vi "measure BT Min Freq.vi"(8 "error in (no error)":errorcluster, 10 "Threshold Level":dbl, 11 "SA Measurement in":refnum<class "SA Measurement.lvclass">) -> (0 "error out":errorcluster, 3 "SA Measurement out":refnum<class "SA Measurement.lvclass">)   [LabVIEW 2023, in "Spectrum Analyzer.lvlib" / "SA Measurement.lvclass"]
uses:
  SA Measurement.lvclass
  SA Measurement.lvclass/SA Measurement.ctl
  TYPE DEFINITION/Keysight 9020A/TYPE Measurement Preset.ctl
  Spectrum Analyzer.lvlib
  TYPE DEFINITION/TYPE RBW and VBW Select.ctl
  Interface_Spectrum/Interface_Spectrum.lvclass
  <vilib>/Utility/file.llb/Read Delimited Spreadsheet (string).vi
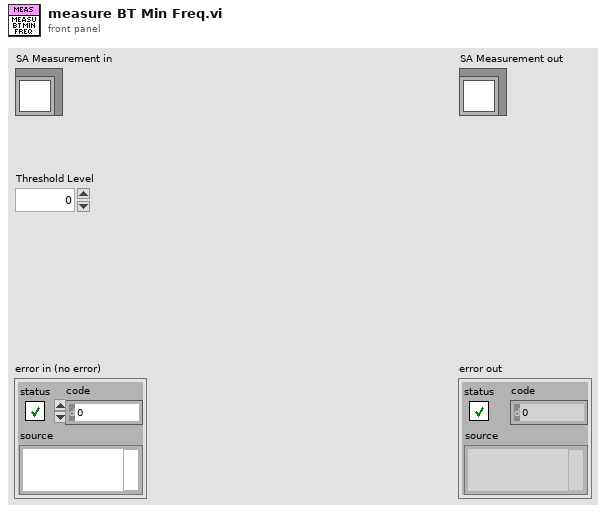
[diagram p1: front panel]
types:
  T1 = typedef "Spectrum Analyzer.lvlib/TYPE RBW and VBW Select.ctl" = enum16{"Res BW", "Video BW"}
  T2 = typedef "Spectrum Analyzer.lvlib/TYPE Measurement Preset.ctl" = enum16{"Sweep SA Mode", "Channel Power", "Occupied BW", "ACP", "Spurious Emission", "Spurious Emission Mask", "Burst Power (Transmit Power)"}
  T3 = typedef "Spectrum Analyzer.lvlib/TYPE Reference Level and Atten Param.ctl" = cluster{"Reference Level":dbl, "Atten":i32, "Atten Auto?":bool, "Reference Level Offset":dbl}
  T4 = typedef "Spectrum Analyzer.lvlib/TYPE Display Trace Mode Select.ctl" = enum16{"Clear Write", "Max Hold", "Min Hold", "Average", "View"}
  T5 = typedef "Spectrum Analyzer.lvlib/TYPE Detect Mode Select.ctl" = enum16{"Det Auto (Normal)", "Auto Peak", "Positive Peak", "Negative Peak", "Sample", "RMS", "Average", "Quasipeak", "CISPR Average", "RMS Average"}
  T6 = cluster{"Trace Mode":T4, "Detector Type":T5, "Detect Auto?":bool}[]
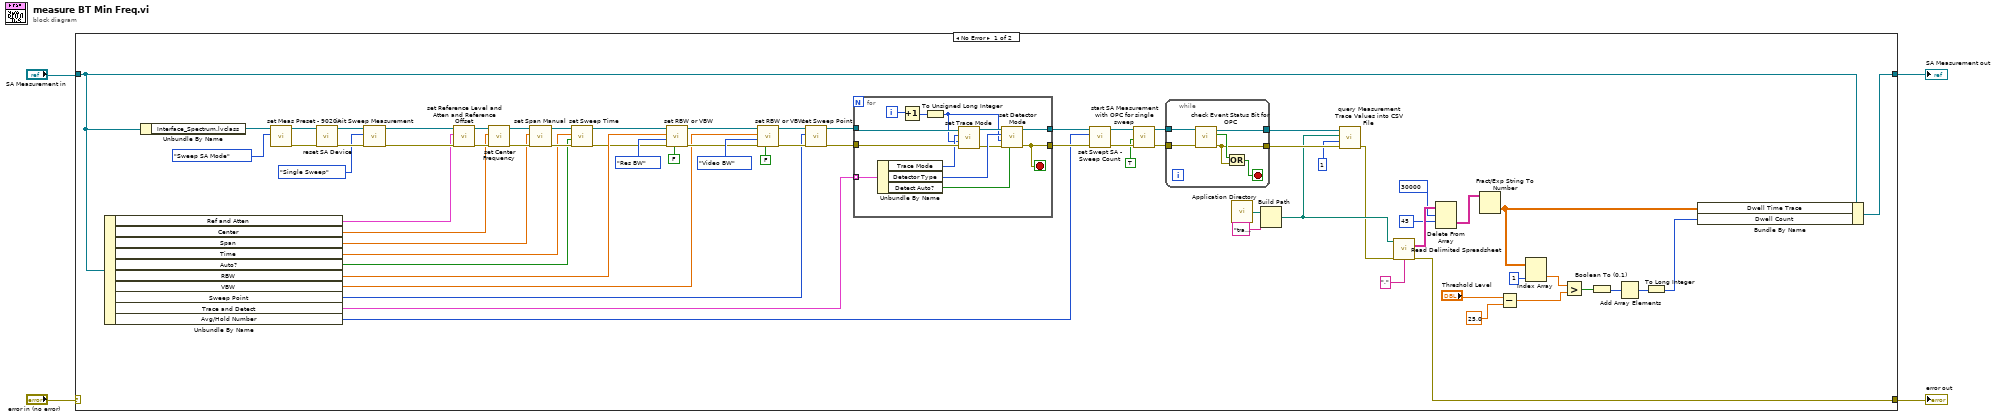
[diagram p0: block diagram]
diagram:
  n1 = case shown="No Error" "error in (no error)" {
    selector: "error in (no error)" -> [_ w94]
    tunnel: [w5 w94] -> w1
    tunnel: [w40 w93] -> w2
    tunnel: "SA Measurement in" -> [w41 w93]
    frame No Error {
      n2 = Unbundle By Name(w41) -> ("Ref and Atten"=w64:T3, "Center"=w37:dbl, "Span"=w34:dbl, "Time"=w31:dbl, "Auto?"=w30:bool, "RBW"=w57:dbl, "VBW"=w56:dbl, "Sweep Point"=w53:u32, "Trace and Detect"=w50:T6, "Avg/Hold Number"=w47:u32)
      n3 = Unbundle By Name(w41) -> ("Interface_Spectrum.lvclass"=w73:refnum<class "Interface_Spectrum.lvclass">)
      n4 = call-dynamic "set Meas Preset - 9020A.vi"("Measurement Preset"=TYPE_Measurement_Preset."Sweep SA Mode", "Interface_Spectrum in"=w73) -> ("error out"=w70:errorcluster, "Interface_Spectrum out"=w71:refnum<class "Interface_Spectrum.lvclass">)  [unwired: 8 in]
      n5 = call-dynamic "reset SA Device.vi"("error in (no error)"=w70, "Interface_Spectrum in"=w71) -> ("error out"=w68:errorcluster, "Interface_Spectrum out"=w69:refnum<class "Interface_Spectrum.lvclass">)  [unwired: 8 in]
      n6 = call-dynamic "init Sweep Measurement.vi"("error in (no error)"=w68, "Sweep Measurement Mode"=enum16{"Single Sweep", "Continuous Sweep"}."Single Sweep", "Interface_Spectrum in"=w69) -> ("error out"=w65:errorcluster, "Interface_Spectrum out"=w66:refnum<class "Interface_Spectrum.lvclass">)  [unwired: 7 in]
      n7 = call-dynamic "set Reference Level and Atten and Reference Offset.vi"("error in (no error)"=w65, "Reference Level, Atten, Reference Offset"=w64, "Interface_Spectrum in"=w66) -> ("error out"=w38:errorcluster, "Interface_Spectrum out"=w39:refnum<class "Interface_Spectrum.lvclass">)  [unwired: 7 in]
      n8 = call-dynamic "set Center Frequency.vi"("error in (no error)"=w38, "Center Frequency (Hz)"=w37, "Interface_Spectrum in"=w39) -> ("error out"=w35:errorcluster, "Interface_Spectrum out"=w36:refnum<class "Interface_Spectrum.lvclass">)  [unwired: 7 in]
      n9 = call-dynamic "set Span Manual.vi"("error in (no error)"=w35, "Span (Hz)"=w34, "Interface_Spectrum in"=w36) -> ("error out"=w32:errorcluster, "Interface_Spectrum out"=w33:refnum<class "Interface_Spectrum.lvclass">)  [unwired: 7 in]
      n10 = call-dynamic "set Sweep Time.vi"("error in (no error)"=w32, "Sweep Time Auto?"=w30, "Sweep Time(sec)"=w31, "Interface_Spectrum in"=w33) -> ("error out"=w28:errorcluster, "Interface_Spectrum out"=w29:refnum<class "Interface_Spectrum.lvclass">)  [unwired: 6 in]
      n11 = call-dynamic "set RBW or VBW.vi"("BW Auto?"=FALSE, "error in (no error)"=w28, "BW Type"=TYPE_RBW_and_VBW_Select."Res BW", "BW Value (Hz)"=w57, "Interface_Spectrum in"=w29) -> ("error out"=w58:errorcluster, "Interface_Spectrum out"=w59:refnum<class "Interface_Spectrum.lvclass">)  [unwired: 5 in]
      n12 = call-dynamic "set RBW or VBW.vi"("BW Auto?"=FALSE, "error in (no error)"=w58, "BW Type"=TYPE_RBW_and_VBW_Select."Video BW", "BW Value (Hz)"=w56, "Interface_Spectrum in"=w59) -> ("error out"=w54:errorcluster, "Interface_Spectrum out"=w55:refnum<class "Interface_Spectrum.lvclass">)  [unwired: 5 in]
      n13 = call-dynamic "set Sweep Point.vi"("error in (no error)"=w54, "Sweep Point"=w53, "Interface_Spectrum in"=w55) -> ("error out"=w51:errorcluster, "Interface_Spectrum out"=w52:refnum<class "Interface_Spectrum.lvclass">)  [unwired: 7 in]
      n14 = for {
        tunnel: w52 -> [w91]
        tunnel: w51 -> [w90]
        tunnel: w50 -> [w92] mode=indexing
        tunnel: [w80] -> w48
        tunnel: [w81] -> w49
        i -> [w89]
        stop <- w80 stop-if-true
        n15 = Unbundle By Name(w92) -> ("Trace Mode"=w87:T4, "Detector Type"=w85:T5, "Detect Auto?"=w82:bool)
        n16 = Increment(x=w89) -> (x+1=w88:i32)
        n17 = To Unsigned Long Integer(number=w88) -> (unsigned 32bit integer=w83:u32)
        n18 = call-dynamic "set Trace Mode.vi"("error in (no error)"=w90, "Trace Index"=w83, "Trace Mode"=w87, "Interface_Spectrum in"=w91) -> ("error out"=w84:errorcluster, "Interface_Spectrum out"=w86:refnum<class "Interface_Spectrum.lvclass">)  [unwired: 6 in]
        n19 = call-dynamic "set Detector Mode.vi"("Detect Auto?"=w82, "error in (no error)"=w84, "Trace Index"=w83, "Detector Type"=w85, "Interface_Spectrum in"=w86) -> ("error out"=w80:errorcluster, "Interface_Spectrum out"=w81:refnum<class "Interface_Spectrum.lvclass">)  [unwired: 5 in]
      }
      n20 = call-dynamic "set Swept SA - Sweep Count.vi"("error in (no error)"=w48, "Sweep Count"=w47, "Interface_Spectrum in"=w49) -> ("error out"=w45:errorcluster, "Interface_Spectrum out"=w46:refnum<class "Interface_Spectrum.lvclass">)  [unwired: 7 in]
      n21 = call-dynamic "start SA Measurement with OPC for single sweep.vi"("error in (no error)"=w45, "with OPC?"=TRUE, "Interface_Spectrum in"=w46) -> ("error out"=w42:errorcluster, "Interface_Spectrum out"=w43:refnum<class "Interface_Spectrum.lvclass">)  [unwired: 7 in]
      n22 = while {
        tunnel: w43 -> [w79]
        tunnel: w42 -> [w78]
        tunnel: [w75] -> w24
        tunnel: [w74] -> w25
        stop <- w76 stop-if-true
        n23 = call-dynamic "check Event Status Bit for OPC.vi"("error in (no error)"=w78, "Interface_Spectrum in"=w79) -> ("error out"=w75:errorcluster, "OPC Bit Changed?"=w77:bool, "Interface_Spectrum out"=w74:refnum<class "Interface_Spectrum.lvclass">)  [unwired: 7 in]
        n24 = Or(x=w77, y=w75) -> (x .or. y?=w76:bool)
      }
      n25 = call <vilib>:"Application Directory.vi"() -> ("Application Directory"=w27:path)
      n26 = Build Path(base path=w27, name or relative path="traceRawdata.csv") -> (appended path=w17:path)
      n27 = call-dynamic "query Measurement Trace Values into CSV File.vi"("error in (no error)"=w24, "Trace Index"=1, "Path"=w17, "Interface_Spectrum in"=w25) -> ("error out"=w16:errorcluster)  [unwired: 6 in, 1 out]
      n28 = call-poly <vilib>:"Read Delimited Spreadsheet.vi"("file path (dialog if empty)"=w17, "error in (no error)"=w16, "delimiter (\\t)"="," ("delimiter (\\t)")) -> ("all rows"=w21:string[][], "error out"=w5:errorcluster)  [unwired: 7 in, 4 out]
      n29 = Delete From Array(array=w21, length=30000, index (row)=45) -> (deleted portion=w18:string[][])  [unwired: 1 in, 1 out]
      n30 = Fract/Exp String To Number(string=w18) -> (number=w6:dbl[][])  [unwired: 3 in, 1 out]
      n31 = Subtract(x="Threshold Level", y=25.0) -> (x-y=w8:dbl)
      n32 = Index Array(array=w6, index (col)=1 ("disabled index (col)")) -> (element=w9:dbl[])  [unwired: 1 in]
      n33 = Greater?(x=w9, y=w8) -> (0:w12:bool[])
      n34 = Boolean To (0,1)(Boolean=w12) -> (0, 1=w11:i16[])
      n35 = Add Array Elements(numeric array=w11) -> (sum=w10:i16)
      n36 = To Long Integer(number=w10) -> (32bit integer=w7:i32)
      n37 = Bundle By Name(cluster=w41, "Dwell Time Trace"=w6, "Dwell Count"=w7) -> (w40:refnum<class "SA Measurement.lvclass">)
    }
    frame Error {
    }
  }
  "error out" <- w1
  "SA Measurement out" <- w2
